vi "Modify Template.vi"(8 "error in":errorcluster, 11 "ILabVIEWFile in":refnum<class "Virtual Instrument.lvclass">) -> (0 "error out":errorcluster, 3 "ILabVIEWFile out":refnum<class "Virtual Instrument.lvclass">)   [LabVIEW 2026, in "Virtual Instrument.lvclass"]
doc: "This method modifies (i.e. adds/removes/replaces elements in the template) to implement the current file."
uses:
  Virtual Instrument.lvclass
  Type Definitions/Parameter Mode--enum.ctl
  Virtual Instrument.lvclass/Virtual Instrument.ctl
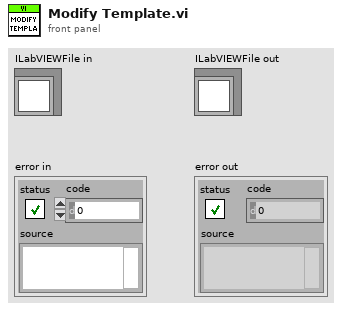
[diagram p1: front panel]
types:
  T1 = typedef "Parameter Mode--enum.ctl" = enum16{"Input", "Output"}
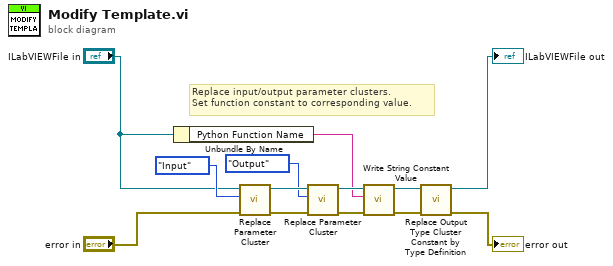
[diagram p0: block diagram]
diagram:
  # "Replace input/output parameter clusters.\nSet function constant to corresponding value."
  n1 = Unbundle By Name("ILabVIEWFile in") -> ("Python Function Name"=w3:string)
  n2 = call "Replace Parameter Cluster.vi"("error in"="error in", "Parameter Mode"=Parameter_Mode--enum."Input", "Virtual Instrument in"="ILabVIEWFile in") -> ("error out"=w12:errorcluster, "Virtual Instrument out"=w8:refnum<class "Virtual Instrument.lvclass">)  [unwired: 7 in]
  n3 = call "Replace Parameter Cluster.vi"("error in"=w12, "Parameter Mode"=Parameter_Mode--enum."Output", "Virtual Instrument in"=w8) -> ("error out"=w11:errorcluster, "Virtual Instrument out"=w5:refnum<class "Virtual Instrument.lvclass">)  [unwired: 7 in]
  n4 = call "Write String Constant Value.vi"("error in"=w11, "Python Function"=w3, "Virtual Instrument in"=w5) -> ("error out"=w10:errorcluster, "Virtual Instrument out"=w2:refnum<class "Virtual Instrument.lvclass">)  [unwired: 7 in]
  n5 = call "Replace Output Type Cluster Constant by Type Definition.vi"("error in"=w10, "Virtual Instrument in"=w2) -> ("error out"=→"error out":errorcluster, "Virtual Instrument out"=→"ILabVIEWFile out":refnum<class "Virtual Instrument.lvclass">)  [unwired: 8 in]
